vi "libssh2_sftp_write.vi"(8 "error in (no error)":errorcluster, 10 "buffer":u8[](array[numeric]), 11 "sftp handle":T1) -> (0 "error out":errorcluster, 2 "bytes acknowledged":i32)   [LabVIEW 2017, in "libssh2.lvlib"]
doc: "Write data to a file handle."
uses:
  libssh2.lvlib
  SFTP Handle Refnum.ctl
  Acquire SFTP.vi
  Release SFTP.vi
  Acquire Session.vi
  Release Session.vi
  Not An SFTP Handle Refnum.vi
  <vilib>/Utility/error.llb/Error Cluster From Error Code.vi
  Global Settings.vi
  Read SFTP Handle Refnum.vi
  Read SFTP Refnum.vi
  Read Session Refnum.vi
  <vilib>/Utility/semaphor.llb/Acquire Semaphore.vi
  <vilib>/Utility/semaphor.llb/Release Semaphore.vi
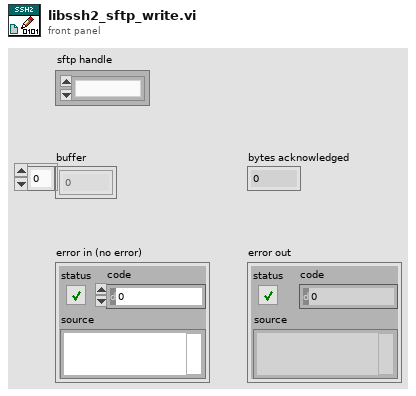
[diagram p1: front panel]
types:
  T1 = typedef "libssh2.lvlib/SFTP Handle Refnum.ctl" = refnum<k1>
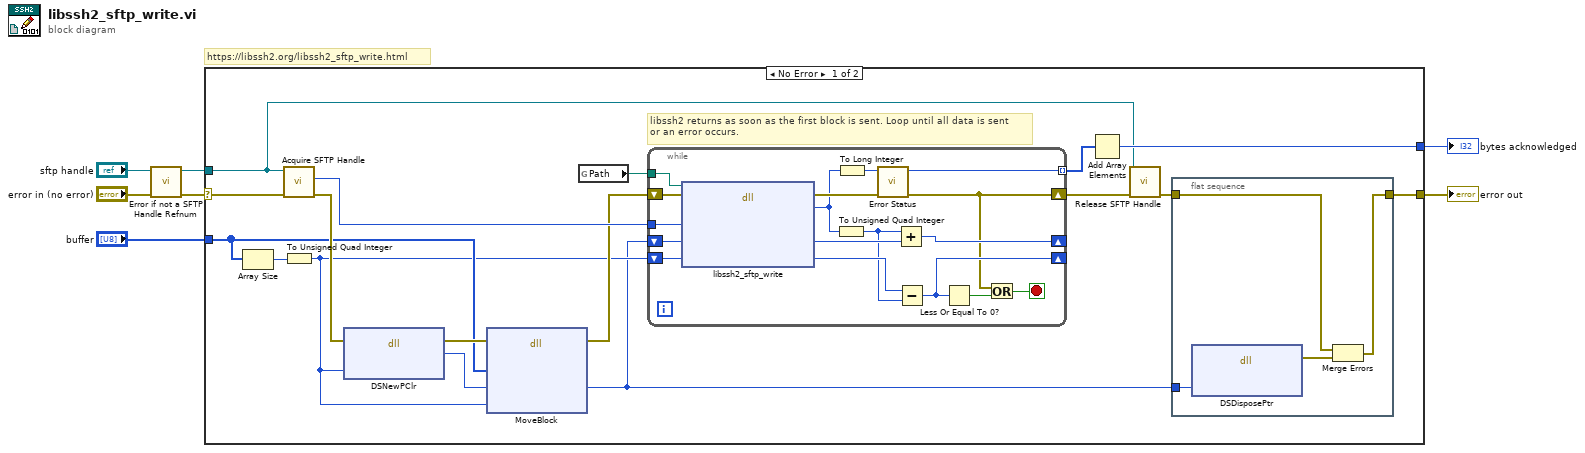
[diagram p0: block diagram]
diagram:
  # "https://libssh2.org/libssh2_sftp_write.html"
  n1 = call "Error if not a SFTP Handle Refnum.vi"("error in (no error)"="error in (no error)", "sftp handle"="sftp handle") -> ("error out"=w6:errorcluster, "sftp handle out"=w5:T1)  [unwired: 8 in]
  n2 = case shown="No Error" w6 {
    selector: w6 -> [w23 w46]
    tunnel: w5 -> [w8 _]
    tunnel: [w14 w46] -> w4
    tunnel: "buffer" -> [w16 _]
    tunnel: [w11 _] -> w2
    frame No Error {
      # "libssh2 returns as soon as the first block is sent. Loop until all data is sent\nor an error occurs."
      n3 = Array Size(array=w16) -> (size(s)=w21:i32)
      n4 = call "Acquire SFTP Handle.vi"("error in (no error)"=w23, "sftp handle"=w8) -> ("error out"=w18:errorcluster, "LIBSSH2_SFTP_HANDLE*"=w22:u64)  [unwired: 8 in]
      n5 = To Unsigned Quad Integer(1:w21) -> (0:w15:u64)
      n6 = dll-call lib="LabVIEW" fn="DSNewPClr"(error in=w18, "size"=w15) -> (error out=w20:errorcluster, "return type"=w19:u64)  [unwired: 3 in, 1 out]
      n7 = dll-call lib="LabVIEW" fn="MoveBlock"(error in=w20, "ps"=w16, "pd"=w19, "size"=w15) -> (error out=w17:errorcluster, "pd"=w13:u64)  [unwired: 5 in, 1 out]
      n8 = global read "Global Settings.vi" "Path"() -> (w24:path)
      n9 = while {
        tunnel: w24 -> [w41]
        tunnel: w22 -> [w40]
        shift-right: [w32] -> _
        shift-left: w13 -> [w37]
        shift-right: [w31] -> _
        shift-left: w15 -> [w38]
        tunnel: [w27] -> w12 mode=indexing
        shift-right: [w29] -> w10
        shift-left: w17 -> [w39]
        stop <- w34 stop-if-true
        n10 = dll-call lib="?" fn="libssh2_sftp_write"(path in=w41, error in=w39, "handle"=w40, "buffer"=w37, "count"=w38) -> (error out=w30:errorcluster, "return value"=w26:i64, "buffer"=w33:u64, "count"=w36:u64)  [unwired: 2 in, 1 out]
        n11 = To Unsigned Quad Integer(1:w26) -> (0:w25:u64)
        n12 = To Long Integer(number=w26) -> (32bit integer=w28:i32)
        n13 = call "Error Status.vi"("error in (no error)"=w30, "return value"=w28) -> ("error out"=w29:errorcluster, "return value out"=w27:i32)  [unwired: 8 in]
        n14 = Add(x=w25, y=w33) -> (x+y=w32:u64)
        n15 = Subtract(x=w36, y=w25) -> (x-y=w31:u64)
        n16 = Less Or Equal To 0?(x=w31) -> (x <= 0?=w35:bool)
        n17 = Or(x=w29, y=w35) -> (x .or. y?=w34:bool)
      }
      n18 = Add Array Elements(numeric array=w12) -> (sum=w11:i32)
      n19 = call "Release SFTP Handle.vi"("error in (no error)"=w10, "sftp handle"=w8) -> ("error out"=w9:errorcluster)  [unwired: 9 in]
      n20 = flat-sequence {
        tunnel: [w43] -> w14
        tunnel: w9 -> [w44]
        tunnel: w13 -> [w45]
        frame #0 {
          n21 = dll-call lib="LabVIEW" fn="DSDisposePtr"("p"=w45) -> (error out=w42:errorcluster)  [unwired: 5 in, 1 out]
          n22 = Merge Errors(w44, w42) -> (w43:errorcluster)
        }
      }
    }
    frame Error {
    }
  }
  "error out" <- w4
  "bytes acknowledged" <- w2
